vi "XML - Get absolute RT Driver VI path for TARGET.vi"(7 "Target Type (Windows)":T1, 10 "CD Template":refnum<class "NIVS_CD Template.lvclass">, 11 "Project Name":string) -> (3 "Relative RT Driver TARGET path":path)   [LabVIEW 2020, in "NIVS_Consolidated_CDW_MetaDataObj.lvclass"]
doc: "Create the absolute path for the RT Driver VI inside the Configuration LLB for the <B>RT Target</B> based on the name and execution mode of the new custom device."
uses:
  NIVS_Consolidated_CDW_MetaDataObj.lvclass
  Build Spec Engine.ctl
  CD Engine lvlib.ctl
  Template Classes/NIVS_CD Template/NIVS_CD Template.lvclass
  CD Engine lvlib.vi
  Build Spec Engine.vi
  Template Classes/NIVS_PPLCD Template/NIVS_PPLCD Template.lvclass
  Target Type.ctl
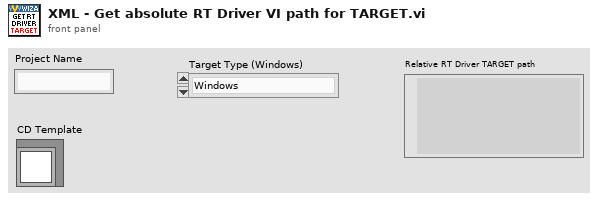
[diagram p1: front panel]
types:
  T1 = typedef "NIVS_Consolidated_CDW_MetaDataObj.lvclass/Target Type.ctl" = enum16{"Windows", "Linux x64"}
  T2 = typedef "NIVS_Consolidated_CDW_MetaDataObj.lvclass/CD Engine lvlib.ctl" = enum16{"LibraryFileName", "LibraryFolderName", "Engine.FolderName", "Engine.Init.FolderName", "Engine.Run.FolderName", "Engine.Shutdown.FolderName", "Types.FolderName", "Engine.RT Driver VI.TemplatePath", "Engine.RT Driver VI.FileName", "Engine.PPL.RT Driver VI_InlineAsync.FileName", "Engine.RTStateVariables.Name", "Engine.PPL.RTStateVariables.Name", "Engine.RTStateVariables.Name.NoExtension", "Engine.Async.NameExtension", "Engine.Async.TemplateName", "Engine.PPL.Async.TemplateName", "Engine.PPL.Async.InitVSGlobals.Name", "Engine.PPL.RT Driver VI_Inline.FileName"}
  T3 = typedef "NIVS_Consolidated_CDW_MetaDataObj.lvclass/Build Spec Engine.ctl" = enum16{"Destinations.LLBWindowsFileName", "Destinations.LLBLinux64FileName", "Destinations.PPLWindowsFileName", "Destinations.PPLLinux64FileName"}
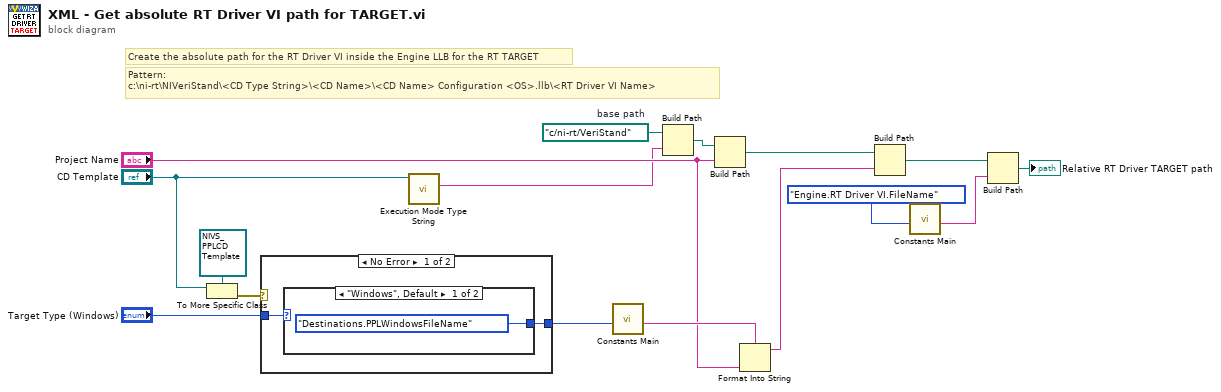
[diagram p0: block diagram]
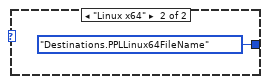
[diagram p2: hidden frame]
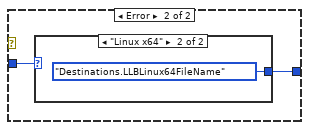
[diagram p3: hidden frame]
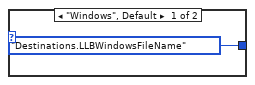
[diagram p4: hidden frame]
diagram:
  w10 = path "c:/ni-rt/VeriStand"  # base path
  # "Create the absolute path for the RT Driver VI inside the Engine LLB for the RT TARGET"
  # "Pattern:\nc:\\ni-rt\\NIVeriStand\\<CD Type String>\\<CD Name>\\<CD Name> Configuration <OS>.llb\\<RT Driver VI Name>"
  n1 = To More Specific Class(target class=refnum<class "NIVS_PPLCD Template.lvclass"> refnum ("NIVS_PPLCD Template.lvclass"), reference="CD Template") -> (error out=w1:errorcluster)  [unwired: 1 in, 1 out]
  n2 = case shown="No Error" w1 {
    tunnel: "Target Type (Windows)" -> [w17 w22]
    tunnel: [w18 w21] -> w11
    frame No Error {
      n3 = case shown="\"Windows\", Default" w17 {
        tunnel: [Build_Spec_Engine."Destinations.PPLWindowsFileName" ("Action") Build_Spec_Engine."Destinations.PPLLinux64FileName" ("Action")] -> w18
        frame "Windows", Default {
        }
        frame "Linux x64" {
        }
      }
    }
    frame Error {
      n4 = case shown="\"Linux x64\"" w22 {
        tunnel: [Build_Spec_Engine."Destinations.LLBWindowsFileName" ("Action") Build_Spec_Engine."Destinations.LLBLinux64FileName" ("Action")] -> w21
        frame "Windows", Default {
        }
        frame "Linux x64" {
        }
      }
    }
  }
  n5 = call-dynamic "Execution Mode Type String.vi"("CD Template"="CD Template") -> ("Execution Mode Type String"=w4:string)  [unwired: 10 in]
  n6 = call-poly "Constants Main.vi"("Action"=w11) -> ("Output"=w13:string)  [unwired: 10 in]
  n7 = Build Path(base path=w10, name or relative path=w4) -> (appended path=w9:path)
  n8 = Build Path(base path=w9, name or relative path="Project Name") -> (appended path=w12:path)
  n9 = Format Into String(format string=w13, "Project Name") -> (resulting string=w14:string)  [unwired: 2 in, 1 out]
  n10 = Build Path(base path=w12, name or relative path=w14) -> (appended path=w7:path)
  n11 = call-poly "Constants Main.vi"("Action"=CD_Engine_lvlib."Engine.RT Driver VI.FileName") -> ("Output"=w6:string)  [unwired: 10 in]
  n12 = Build Path(base path=w7, name or relative path=w6) -> (appended path=→"Relative RT Driver TARGET path":path)
